vi "lvmcp_replace.vi"() -> ()   [LabVIEW 2026]
panel:
  out "error out":errorcluster
  out "reference out":refnum<vi>
  out "Replace":refnum<vi>
  in  "reference":refnum<vi>
  in  "Palette String":string
  in  "Style":u32
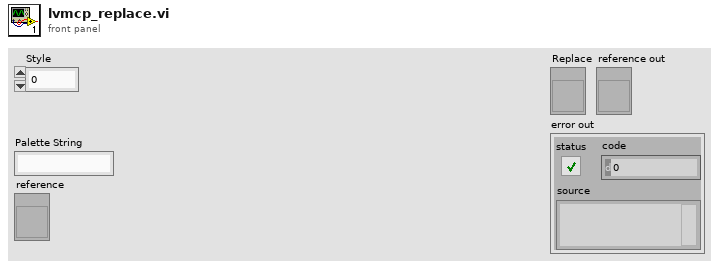
[diagram p1: front panel]
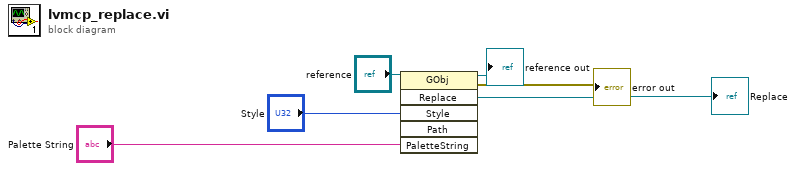
[diagram p0: block diagram]
diagram:
  n1 = invoke class="GObj" method="Replace"(reference="reference", "Style"="Style", "PaletteString"="Palette String") -> (reference out=→"reference out":refnum<vi>, error out=→"error out":errorcluster, "Replace"=→"Replace":refnum<vi>)  [unwired: 3 in, 3 out]
